vi "Parse NSA Call Process Param.vi"(8 "error in (no error)":errorcluster caption="에러 입력(에러 없음)", 10 "JSON string":string, 11 "Instrument Manager 입력":refnum<class "Instrument Manager.lvclass">) -> (0 "error out":errorcluster caption="에러 출력", 1 "NSA Call Process Param":T2, 2 "Call Handover Param LTE":T1, 3 "Instrument Manager 출력":refnum<class "Instrument Manager.lvclass">)   [LabVIEW 2023, in "Instrument Manager.lvclass"]
uses:
  Instrument Manager.lvclass
  Param Definition/NSA Call Process Param.ctl
  Module/ANRITSU Call Box/Type Definition/NR Modulation Type.ctl
  Param Definition/Call Handover Param NSA.ctl
  Call Process Param NSA.ctl
  Instrument Manager.lvclass/Instrument Manager.ctl
  Module/ANRITSU Call Box/ANRITSU Call Box.lvlib
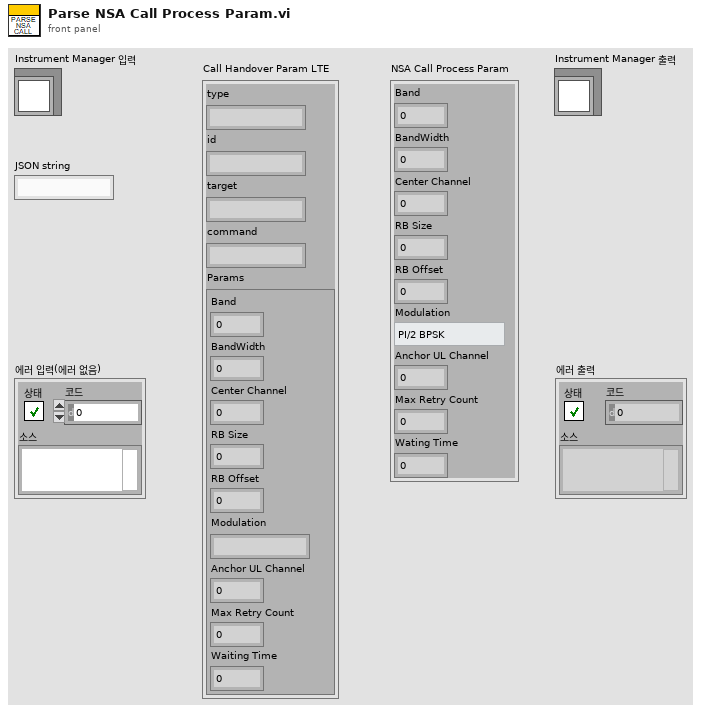
[diagram p1: front panel]
types:
  T1 = typedef "Instrument Manager.lvclass/Call Handover Param NSA.ctl" = cluster{"type":string, "id":string, "target":string, "command":string, "Params":cluster{"Band":u32, "BandWidth":u32, "Center Channel":u32, "RB Size":i32, "RB Offset":i32, "Modulation":string, "Anchor UL Channel":i32, "Max Retry Count":i32, "Waiting Time":i32}}
  T2 = typedef "NSA Call Process Param.ctl" = cluster{"Band":u32, "BandWidth":u32, "Center Channel":u32, "RB Size":i32, "RB Offset":i32, "Modulation":T3, "Anchor UL Channel":i32, "Max Retry Count":i32, "Wating Time":i32}
  T3 = typedef "ANRITSU Call Box.lvlib/NR Modulation Type.ctl" = enum16{"PI/2 BPSK", "QPSK", "16QAM", "64QAM", "256QAM"}
  T4 = typedef "Instrument Manager.lvclass/Call Process Param NSA.ctl" = cluster{"type":string, "id":string, "target":string, "command":string, "Params":cluster{"Band":u32, "BandWidth":u32, "Center Channel":u32, "RB Size":i32, "RB Offset":i32, "Modulation":string, "Anchor UL Channel":i32, "Max Retry Count":i32, "Waiting Time":i32}}
  T5 = cluster{"Band":u32, "BandWidth":u32, "Center Channel":u32, "RB Size":i32, "RB Offset":i32, "Modulation":string, "Anchor UL Channel":i32, "Max Retry Count":i32, "Waiting Time":i32}
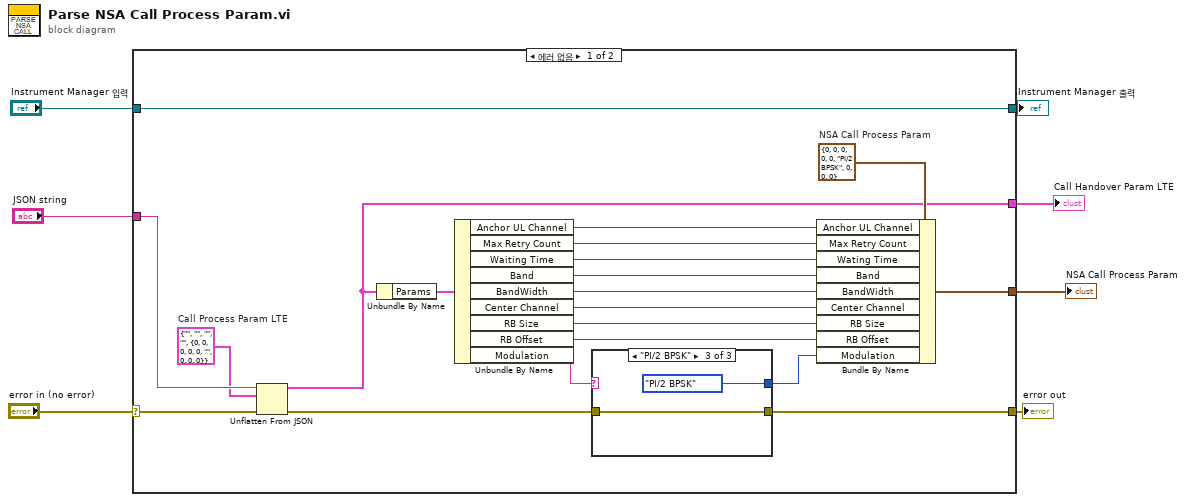
[diagram p0: block diagram]
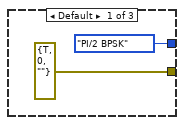
[diagram p2: hidden frame]
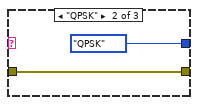
[diagram p3: hidden frame]
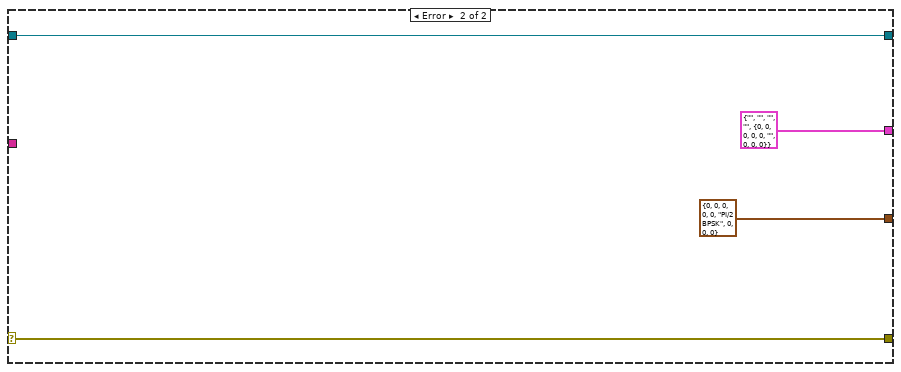
[diagram p4: hidden frame]
diagram:
  n1 = case shown="에러 없음" "error in (no error)" {
    selector: "error in (no error)" -> [w13 w37]
    tunnel: [w11 w37] -> w6
    tunnel: [w27 w36] -> w4
    tunnel: "Instrument Manager 입력" -> [w27 w36]
    tunnel: "JSON string" -> [w12 _]
    tunnel: [w10 T2 {"Band"=0, "BandWidth"=0, "Center Channel"=0, "RB Size"=0, "RB Offset"=0, "Modulation"=enum."PI/2 BPSK", "Anchor UL Channel"=0, "Max Retry Count"=0, "Wating Time"=0} ("NSA Call Process Param")] -> w2
    tunnel: [w9 T4 {"type"="", "id"="", "target"="", "command"="", "Params"={"Band"=0, "BandWidth"=0, "Center Channel"=0, "RB Size"=0, "RB Offset"=0, "Modulation"="", "Anchor UL Channel"=0, "Max Retry Count"=0, "Waiting Time"=0}} ("Call Handover Param LTE")] -> w1
    frame No Error {
      w8 = T4 {"type"="", "id"="", "target"="", "command"="", "Params"={"Band"=0, "BandWidth"=0, "Center Channel"=0, "RB Size"=0, "RB Offset"=0, "Modulation"="", "Anchor UL Channel"=0, "Max Retry Count"=0, "Waiting Time"=0}}  # Call Process Param LTE
      w14 = T2 {"Band"=0, "BandWidth"=0, "Center Channel"=0, "RB Size"=0, "RB Offset"=0, "Modulation"=enum."PI/2 BPSK", "Anchor UL Channel"=0, "Max Retry Count"=0, "Wating Time"=0}  # NSA Call Process Param
      n2 = Unflatten From JSON(JSON string=w12, type and defaults=w8, error in (no error)=w13) -> (value=w9:T4, error out=w23:errorcluster)  [unwired: 4 in]
      n3 = Unbundle By Name(w9) -> ("Params"=w15:T5)
      n4 = Unbundle By Name(w15) -> ("Anchor UL Channel"=w26:i32, "Max Retry Count"=w25:i32, "Waiting Time"=w17:i32, "Band"=w18:u32, "BandWidth"=w19:u32, "Center Channel"=w20:u32, "RB Size"=w21:i32, "RB Offset"=w22:i32, "Modulation"=w16:string)
      n5 = case shown="\"PI/2 BPSK\"" w16 {
        tunnel: w23 -> [_ w30 w32]
        tunnel: [NR_Modulation_Type."PI/2 BPSK" ("Modulation") NR_Modulation_Type."QPSK" ("Modulation") NR_Modulation_Type."PI/2 BPSK" ("Modulation")] -> w24
        tunnel: [errorcluster {"status"=TRUE, "code"=0, "source"=""} ("error out") w30 w32] -> w11
        frame Default {
        }
        frame "QPSK" {
        }
        frame "PI/2 BPSK" {
        }
      }
      n6 = Bundle By Name(cluster=w14, "Anchor UL Channel"=w26, "Max Retry Count"=w25, "Wating Time"=w17, "Band"=w18, "BandWidth"=w19, "Center Channel"=w20, "RB Size"=w21, "RB Offset"=w22, "Modulation"=w24) -> (w10:T2)
    }
    frame Error {
    }
  }
  "error out" <- w6
  "Instrument Manager 출력" <- w4
  "NSA Call Process Param" <- w2
  "Call Handover Param LTE" <- w1
